vi "CIF Subscriber from Refnum.vi"(3 "CIF Subscriber Refnum":T1 {"refnum" format="%.0x"}) -> (5 "CIF Subscriber U64":u64)   [LabVIEW 2021, in "Iceoryx.lvlib"]
uses:
  Iceoryx.lvlib
  Typedef/CIF Subscriber Refnum.ctl
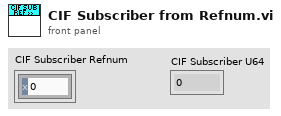
[diagram p1: front panel]
types:
  T1 = typedef "Iceoryx.lvlib/CIF Subscriber Refnum.ctl" = cluster{"refnum":u64}
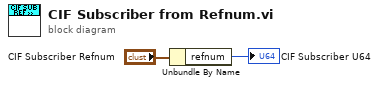
[diagram p0: block diagram]
diagram:
  n1 = Unbundle By Name("CIF Subscriber Refnum") -> ("refnum"=→"CIF Subscriber U64":u64)
